vi "TDM Transmit Receive Test.vi"(6 "ready for output":bool, 7 "transfer":bool, 9 "input valid":bool, 10 "transfer length":u8=32, 11 "sample in":u32=2571108608) -> (1 "output valid":bool, 2 "signals out":cluster{"clock":bool, "sync":bool, "sdata":bool}, 3 "sample out":u32, 4 "ready for input":bool)   [LabVIEW 2013]
uses:
  <vilib>/Platform/TimedLoop/XDataNode/timing_clust.ctl
  <vilib>/Platform/TimedLoop/XDataNode/nitl_modes.ctl
  <vilib>/Platform/TimedLoop/XDataNode/wakeup.ctl
  Source/Controls/transmitter configuration.ctl
  Source/Controls/sync modes.ctl
  Source/Controls/receiver configuration.ctl
  <vilib>/rvi/Emulation/niFpgaSctlEmulationGetInTimedLoop.vi
  <vilib>/rvi/Emulation/niFpgaEmulationReportErrorSimple.vi
  <vilib>/rvi/Emulation/niFpgaGetClockAttributes.vi
  <vilib>/rvi/Emulation/niFpgaCriticalErrorInLSC.vi
  <vilib>/Platform/TimedLoop/XDataNode/XDataNode.xnode
  <vilib>/Platform/TimedLoop/XDataNode/XDNodeRunTimeDep.lvlib
  Source/I2S-TDM.lvlib
panel:
  in  "channel count":u8=2
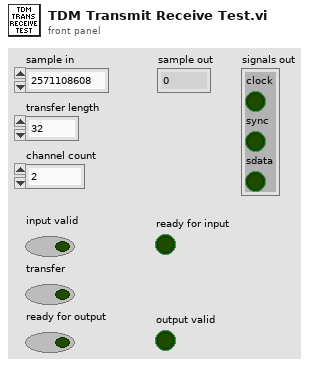
[diagram p1: front panel]
types:
  T1 = typedef "XDNodeRunTimeDep.lvlib/timing_clust.ctl" = cluster{"Expected End [f-1]":u64, "Actual End [f-1]":u64, "Finished Late? [f-1]":bool, "Expected End [i-1]":u64, "Actual End [i-1]":u64, "Finished Late? [i-1]":bool, "Expected Start [i]":u64, "Actual Start [i]":u64, "Expected Start [f]":u64, "Actual Start [f]":u64, "Source Name":string, "Structure Name":string, "Period":i64, "Deadline":i64, "Offset":i64, "Start":i64, "Priority":i32, "Timeout":i32, "Mode":T2, "Wakeup Reason":T3, "Error":errorcluster, "Source Type":string, "Secondary Source Type":string, "Global End Time":u64, "Global Start Time":u64, "Frame Duration":u64, "Iteration Duration":u64, "Assigned CPU":i32, "I/O Scan Engine Mode":u32}
  T2 = typedef "XDNodeRunTimeDep.lvlib/nitl_modes.ctl" = enum32{"No Change", "Process missed periods, maintain original phase", "Discard missed periods, maintain original phase", "Process missed periods, ignore original phase", "Discard missed periods, ignore original phase"}
  T3 = typedef "XDNodeRunTimeDep.lvlib/wakeup.ctl" = enum32{"Normal", "Aborted", "Asynchronous wakeup", "Timing source error", "Timed loop error", "Timeout"}
  T4 = typedef "I2S-TDM.lvlib/sync modes.ctl" = enum16{"TDM - Sample Clock", "TDM - Pre-Start Pulse"}
  T5 = typedef "I2S-TDM.lvlib/receiver configuration.ctl" = cluster{"number of channels":u8, "bits per channel":u8, "data sample edge":enum16{"rising", "falling"}, "frame start delay":u8, "inverted sync":bool}
  T6 = typedef "I2S-TDM.lvlib/transmitter configuration.ctl" = cluster{"number of channels":u8, "bits per channel":u8, "data set edge":enum16{"rising", "falling"}, "sync mode":T4, "invert sync":bool}
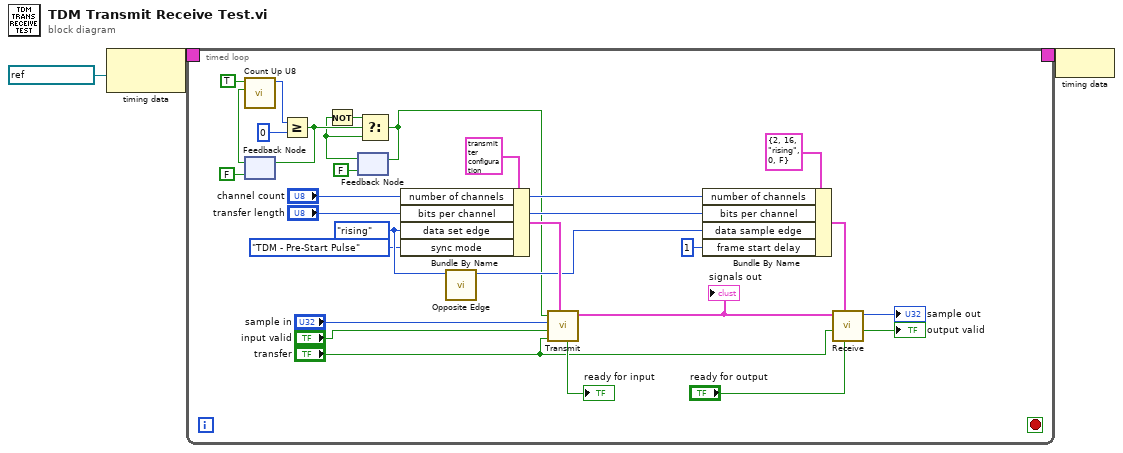
[diagram p0: block diagram]
diagram:
  n1 = node-c288(refnum<k21> "24.576MHz" ("Source Name")) -> (w3:T1)
  n2 = timed-loop {
    timing: w3 -> [_]
    timing-out: [_] -> w2
    stop <- _ stop-if-true
    w19 = enum16{"rising", "falling"}."rising" ("Bit Set Edge")
    n3 = feedback #1(FALSE) -> (w11:bool)
    n4 = call "Count Up U8.vi"("reset (F)"=w11, "increment"=TRUE) -> ("count"=w13:u8)  [unwired: 9 in]
    n5 = Greater Or Equal?(x=w13, y=u8 0) -> (x >= y?=w16:bool)
    n6 = feedback-in #1(w16) -> ()
    n7 = feedback #2(FALSE) -> (w15:bool)
    n8 = Not(x=w15) -> (.not. x?=w9:bool)
    n9 = Select(t=w9, s=w16, f=w15) -> (s? t:f=w8:bool)
    n10 = feedback-in #2(w8) -> ()
    n11 = Bundle By Name(cluster=T6 {"number of channels"=2, "bits per channel"=16, "data set edge"=enum."falling", "sync mode"=enum."TDM - Sample Clock", "invert sync"=FALSE} ("Configuration"), "number of channels"="channel count", "bits per channel"="transfer length", "data set edge"=w19, "sync mode"=sync_modes."TDM - Pre-Start Pulse") -> (w20:T6)
    n12 = call "Opposite Edge.vi"("edge in"=w19) -> ("opposite edge out"=w18:enum16{"rising", "falling"})  [unwired: 10 in]
    n13 = call "Transmit.vi"("configuration"=w20, "transmit"="transfer", "input valid"="input valid", "sample"="sample in", "clock in"=w8) -> ("signals out"=w27:cluster{"clock":bool, "sync":bool, "sdata":bool}, "ready for input"=→"ready for input":bool)  [unwired: 5 in]
    "signals out" <- w27
    n14 = Bundle By Name(cluster=T5 {"number of channels"=2, "bits per channel"=16, "data sample edge"=enum."rising", "frame start delay"=0, "inverted sync"=FALSE} ("configuration"), "number of channels"="channel count", "bits per channel"="transfer length", "data sample edge"=w18, "frame start delay"=u8 1 ("frame sync delay")) -> (w6:T5)
    n15 = call "Receive.vi"("ready for output"="ready for output", "configuration"=w6, "receive"="transfer", "signals in"=w27) -> ("output valid"=→"output valid":bool, "sample"=→"sample out":u32)  [unwired: 6 in]
  }
  n16 = node-c288(w2) -> ()
